vi "Image Marked Areas.vi"(7 "Calling VI Ref":refnum<vi>) -> ()   [LabVIEW 2016]
uses:
  <vilib>/Utility/miscctls.llb/LVPointTypeDef.ctl
  IMA Type Defs/IMA Actions.ctl
  Orca Flash Capture Manager/Orca Flash Capture Manager Controls/Orca Flash Capture Notifier Type.ctl
  Orca Flash Capture Manager/Orca Flash Capture Manager Controls/Orca Flash Capture Actions.ctl
  Orca Flash Capture Manager/Orca Flash Capture Manager Controls/Orca Flash Capture Switch Line Scan Modes.ctl
  Hardware Configuration/Hardware Configuration Controls/Device Function.ctl
  Hardware Configuration/Hardware Configuration Controls/Device Type.ctl
  IMA Type Defs/IMA Marked Positions.ctl
  Wide Field Drift Correction/WFDC Controls/WFDC Notifier Element.ctl
  Wide Field Drift Correction/WFDC Controls/WFDC Actions.ctl
  <vilib>/vision/Image Controls.llb/IMAQ Image.ctl
  Wide Field Drift Correction/WFDC Controls/WFDC External Sync.ctl
  Wide Field Drift Correction/WFDC Controls/WFDC Cycle Pause.ctl
  Wide Field Drift Correction/WFDC Controls/WFDC Status.ctl
  Device Library/Stages/Stages Controls/Stage Actions.ctl
  <vilib>/Utility/error.llb/whitespace.ctl
panel:
  in  "Capture":bool
  in  "Clear All":bool
  in  "Clear Selected":bool
  in  "Mark Point":bool
  in  "Marked Positions":i32(listbox)
  in  "Quit":bool
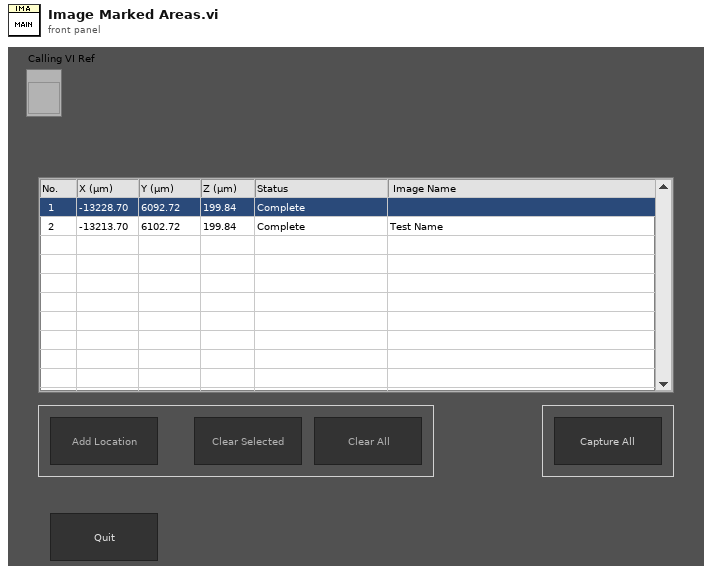
[diagram p1: front panel]
types:
  T1 = typedef "Orca Flash Capture Notifier Type.ctl" = cluster{"Actions":T2, "Running?":bool, "Preview Exposure (s)":dbl, "Capture Exposure (s)":dbl, "Cycles":u16, "Frames":u32, "No. of Z Steps":u16, "Z Step Size (µm)":dbl, "Base Path":path, "Init Z Position (µm)":dbl, "Lasers Lines":string[], "Save Path":path, "Line Scan?":bool, "Line Scan Mode":T3, "Collect Metadata?":bool, "channelCode":u8, "setupName":string}
  T2 = typedef "Orca Flash Capture Actions.ctl" = enum16{"Idle", "Live Preview", "Capture", "Check File Name", "Laser On", "Laser Off", "Open Shutters", "Close Shutters", "Set Exposure Time", "Start Acquisition", "Update SubFolder", "Write Metadata", "Setup", "Camera", "Switch", "Step", "Cycle", "External Cycle Sync", "Abort", "Quit"}
  T3 = typedef "Orca Flash Capture Switch Line Scan Modes.ctl" = enum32{"Automatic", "Use Presets", "Manual"}
  T4 = typedef "IMA Actions.ctl" = enum16{"Add Position", "Update Saved", "Remove Position", "Start Capture", "Move to Position", "Update Name", "Capture", "Switch", "Clear All", "Abort", "Exit Loop", "Quit"}
  T5 = enum16{"Always On", "Always Off", "Off While Running"}
  T6 = typedef "LVPointTypeDef.ctl" = cluster{"Horizontal":i16, "Vertical":i16}
  T7 = enum8{"Enabled", "Disabled", "Disabled and Grayed Out"}
  T8 = typedef "Device Function.ctl" = enum16{"Primary", "Secondary", "Overview", "Wide Field Drift Correction", "642 nm Excitation", "560 nm Excitation", "940 nm Excitation", "546 nm Excitation", "488 nm Excitation", "405 nm Excitation", "Objective Drift Correction", "4Pi Objective Lock", "Objective XY", "Objective Z", "Sample XY", "Sample Coarse Z", "Sample Z", "4Pi Lower", "4Pi Upper", "Mojo", "Adj Cavity", "Line Scanning", "Alert"}
  T9 = typedef "Device Type.ctl" = enum16{"AOTF", "Camera", "Deformable Mirror", "Laser", "Shutter", "Stage", "Waveform", "FPGA", "Email", "Filter Wheel"}
  T10 = typedef "WFDC External Sync.ctl" = cluster{"Cycle Sync":T11, "Z Offset":dbl, "WFDC Status":T12}
  T11 = typedef "WFDC Cycle Pause.ctl" = enum16{"Pause Requested", "Paused", "Resume Requested", "Resumed"}
  T12 = typedef "WFDC Status.ctl" = enum16{"Idle", "Busy", "DC Active", "Error", "Canceled"}
  T13 = typedef "WFDC Notifier Element.ctl" = cluster{"WFDC Actions":T14, "Initial XYZ Positions":dbl[], "Ref Images":T15[], "Calibration (slope, inter)":dbl[], "Log Drift?":bool, "Save WF Images?":bool, "Drift Image File Ref":refnum<file>, "Drift Positions File Ref":refnum<file>, "Base Path":path, "Latest Scan Path":path, "Error":errorcluster}
  T14 = typedef "WFDC Actions.ctl" = enum16{"Error Check", "Remote Start", "Find Focus", "Pre Correct Z", "Pre Correct XY", "Setup New DC", "Setup Camera", "Get Ref Images", "Calc Calibration", "Setup Data Log", "Switch Tabs", "Get Drift / Correct Z", "Correct XY Drift", "Start Cycle", "Stop DC", "Abort Remote", "Exit Loop", "Set Error", "Generate Calibration", "Quit"}
  T15 = typedef "IMAQ Image.ctl" = refnum<image>
  T16 = typedef "IMA Marked Positions.ctl" = cluster{"XYZ Positions":string[][], "File Paths":string[]}
  T17 = enum32{"Invalid", "Standard", "Closed", "Hidden", "Minimized", "Maximized"}
  T18 = typedef "Stage Actions.ctl" = enum16{"Get Position", "MVR", "MOVE", "HALT", "ONTARGET", "ERROR", "REFERENCE", "INIT", "VELOCITY", "STATUS", "EXIT", "HOME", "ZEROPOS", "NANOPOS", "ANALOG", "QUIT"}
  T19 = typedef "whitespace.ctl" = u16
  T20 = typedef "LVRectTypeDef.ctl" = cluster{"Left":i16, "Top":i16, "Right":i16, "Bottom":i16}
  T21 = typedef "LVBoundsTypeDef.ctl" = cluster{"Width":u32, "Height":u32}
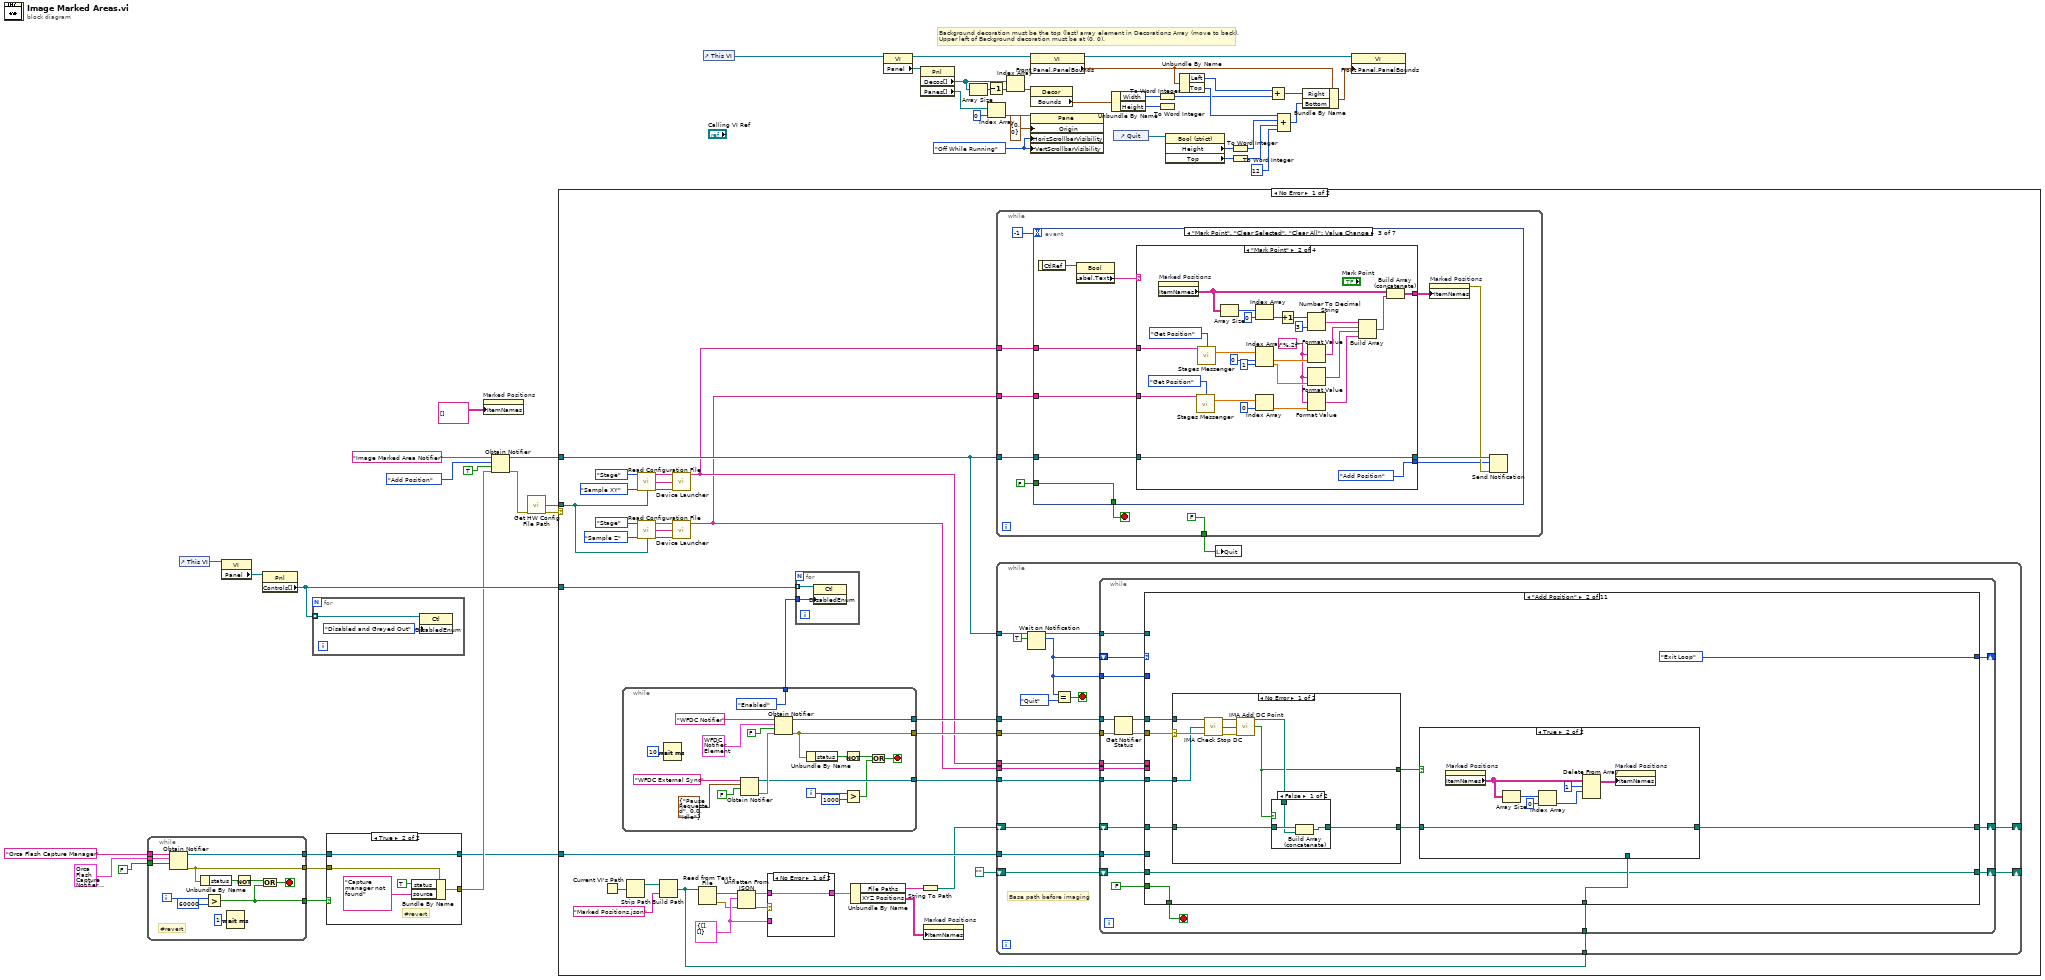
[diagram p0: block diagram]
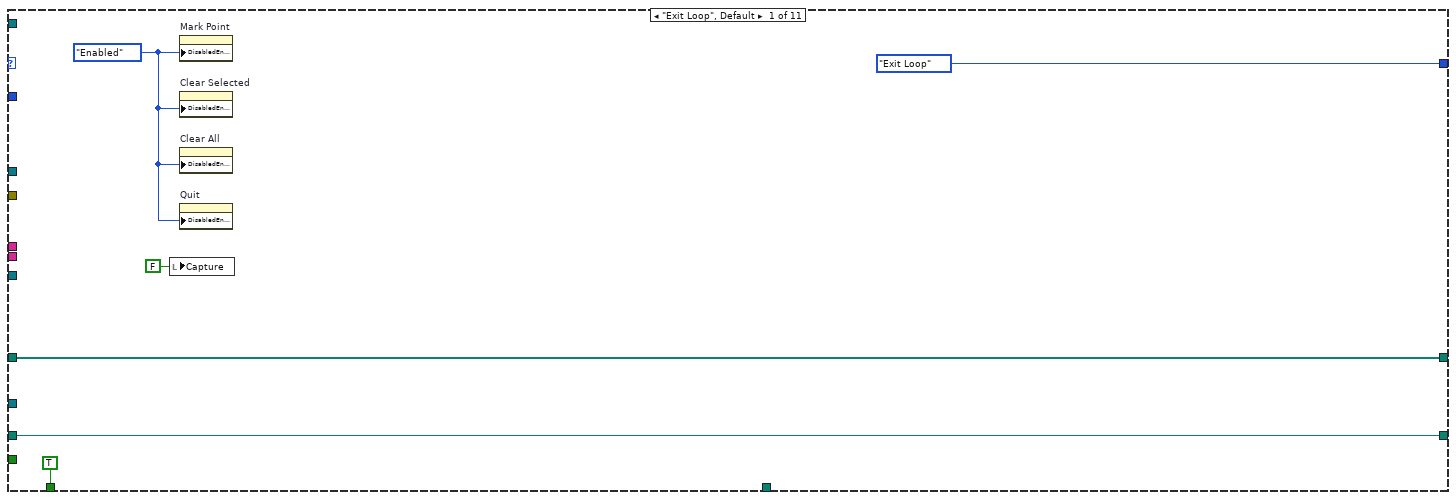
[diagram p4: hidden frame]
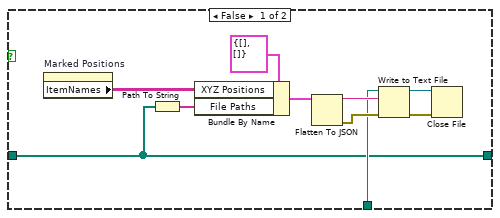
[diagram p5: hidden frame]
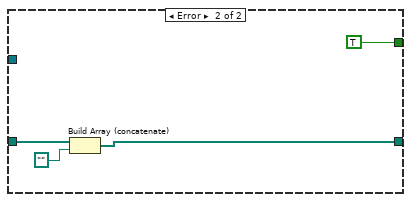
[diagram p7: hidden frame]
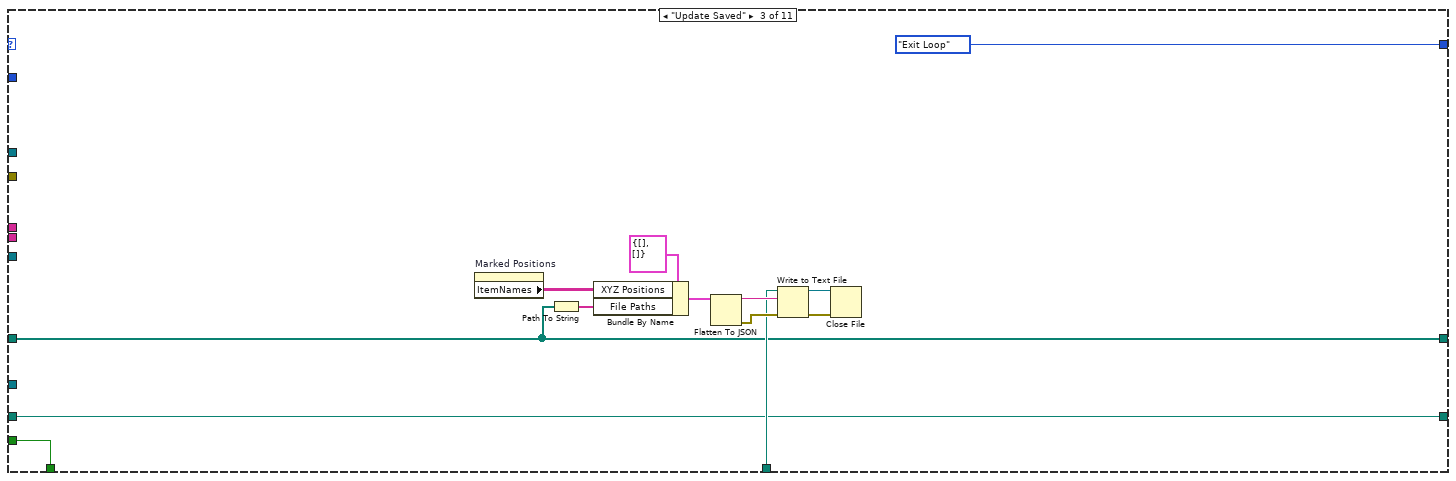
[diagram p8: hidden frame]
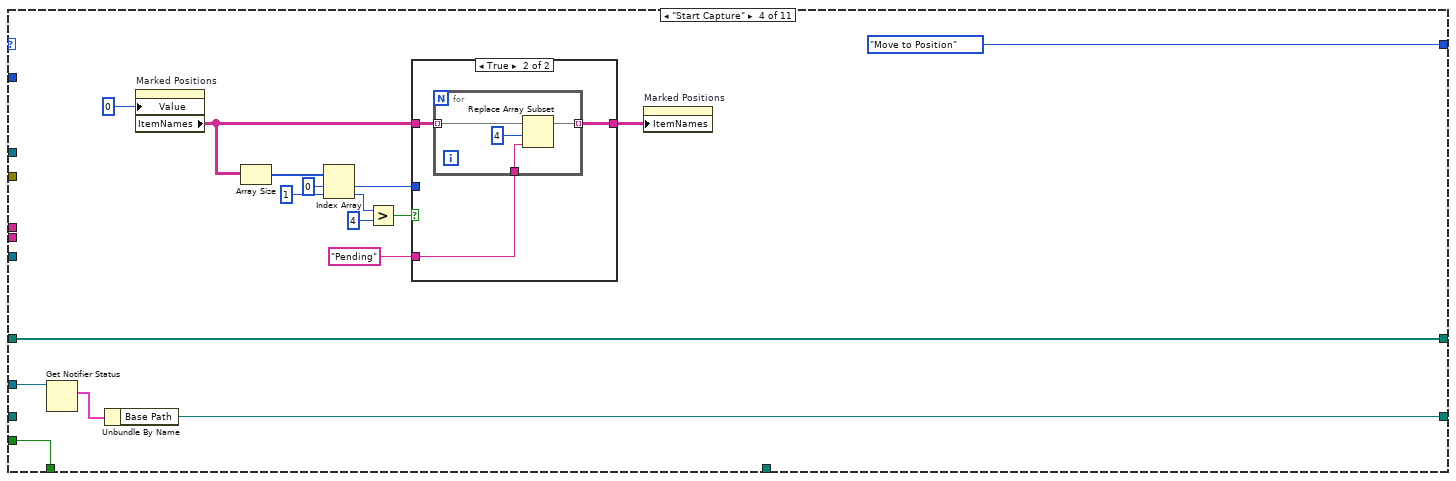
[diagram p9: hidden frame]
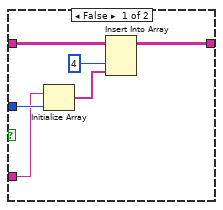
[diagram p10: hidden frame]
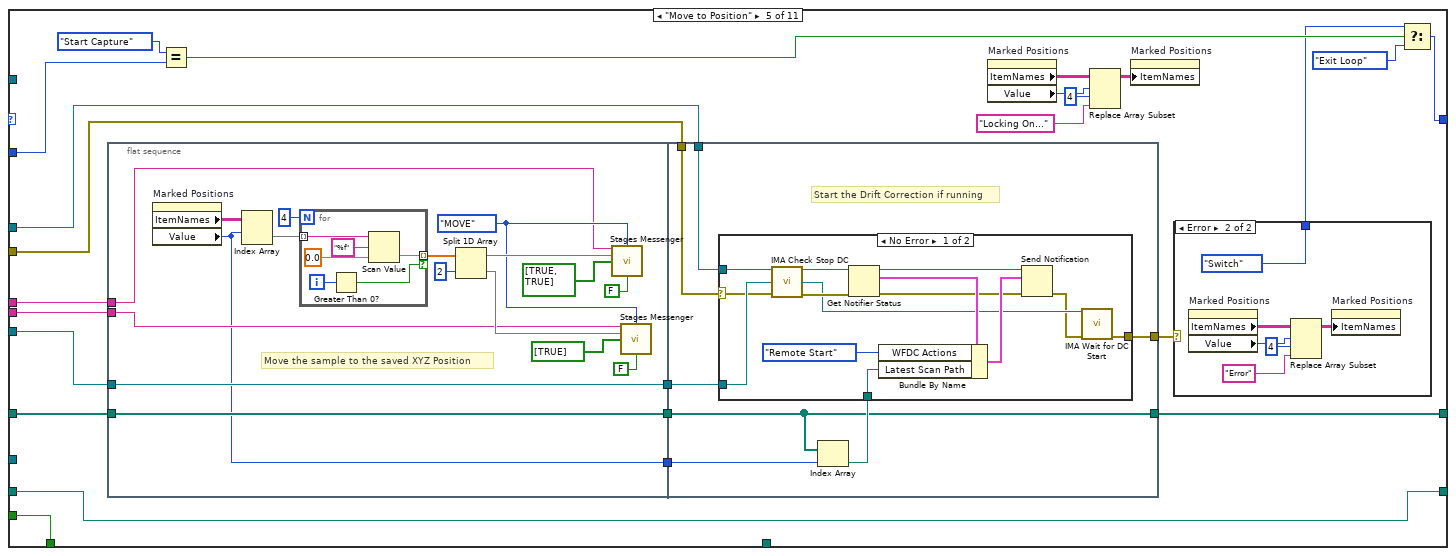
[diagram p11: hidden frame]
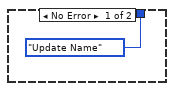
[diagram p12: hidden frame]
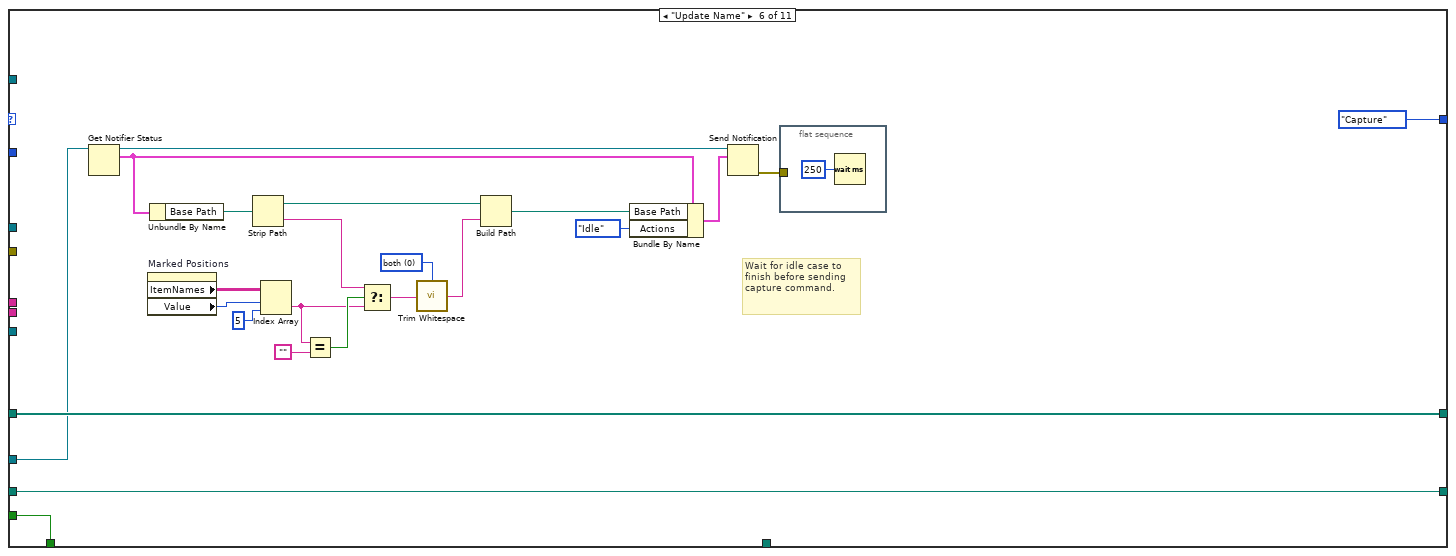
[diagram p14: hidden frame]
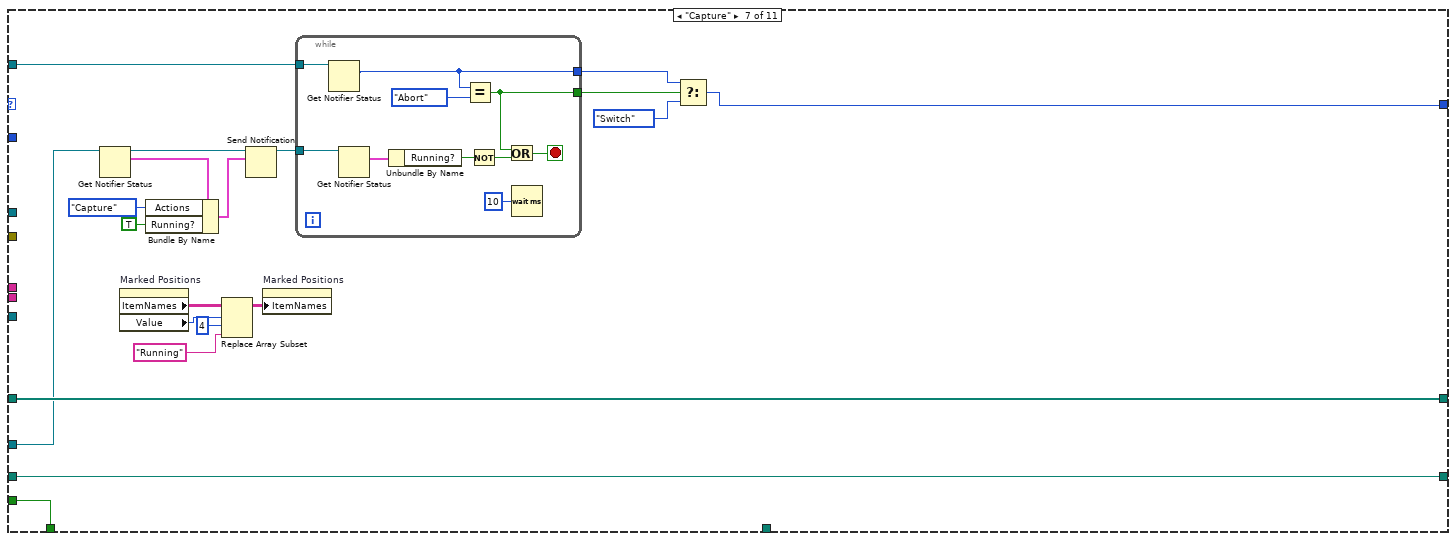
[diagram p15: hidden frame]
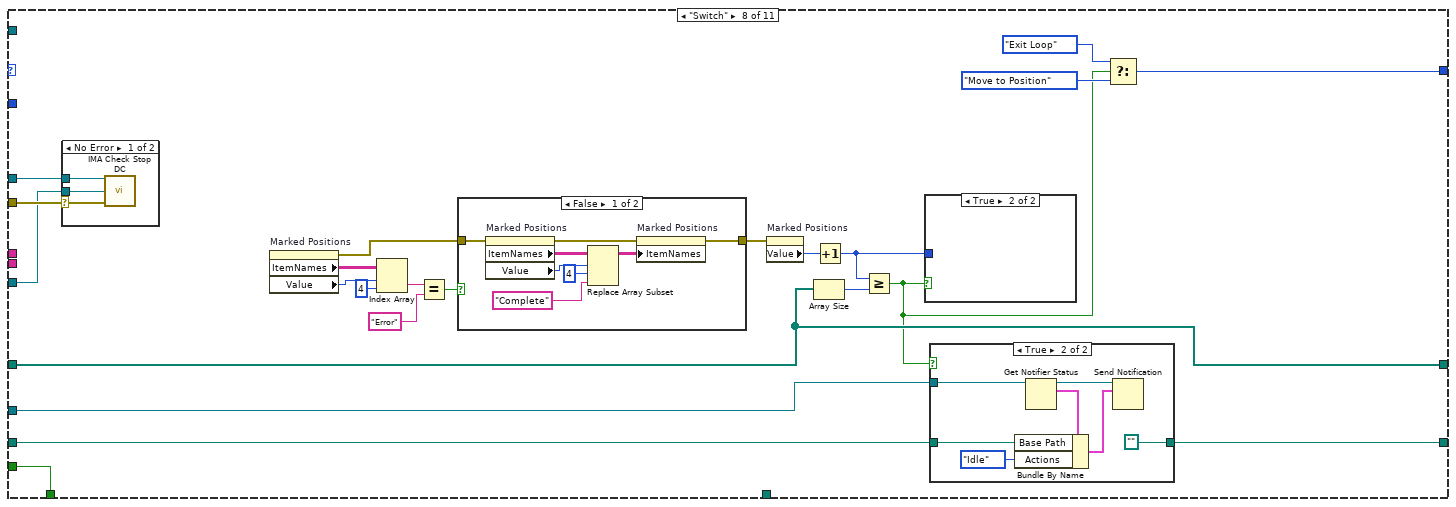
[diagram p16: hidden frame]
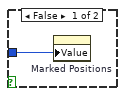
[diagram p20: hidden frame]
diagram:
  w29 = T5."Off While Running" ("Vertical Scrollbar Visibility")
  # "Background decoration must be the top (last) array element in Decorations Array (move to back).\nUpper left of Background decoration must be at (0, 0)."
  n1 = while {
    tunnel: FALSE ("create if not found? (T)") -> [w60]
    tunnel: "Orca Flash Capture Manager" ("name (unnamed)") -> [w59]
    tunnel: T1 {"Actions"=enum."Live Preview", "Running?"=FALSE, "Preview Exposure (s)"=0.1, "Capture Exposure (s)"=0.1, "Cycles"=1, "Frames"=0, "No. of Z Steps"=0, "Z Step Size (µm)"=0.0, "Base Path"=path "", "Init Z Position (µm)"=0.0, "Lasers Lines"=[], "Save Path"=path "", "Line Scan?"=FALSE, "Line Scan Mode"=enum."Automatic", "Collect Metadata?"=FALSE, "channelCode"=0, "setupName"=""} ("4Pi Capture Notifier Type") -> [w58]
    tunnel: [w54] -> w4
    tunnel: [w51] -> w5
    tunnel: [w49] -> w3
    i -> [w57]
    stop <- w50 stop-if-true
    # "#revert"
    n2 = Obtain Notifier(name (unnamed)=w59, notification data type=w58, create if not found? (T)=w60) -> (notifier out=w54:refnum<notifier>, error out=w49:errorcluster)  [unwired: 1 in, 1 out]
    n3 = Unbundle By Name(w49) -> ("status"=w53:bool)
    n4 = Greater?(x=w57, y=60000) -> (0:w51:bool)
    n5 = Wait (ms)(milliseconds to wait=u32 1) -> ()  [unwired: 1 out]
    n6 = Not(x=w53) -> (.not. x?=w52:bool)
    n7 = Or(x=w52, y=w51) -> (x .or. y?=w50:bool)
  }
  n8 = control-ref of="This VI"() -> (w11:refnum<vi>)
  n9 = property class="VI"(reference=w11) -> ("Panel"=w10:refnum<vi>)  [unwired: 1 in, 2 out]
  n10 = property class="Pnl"(reference=w10) -> ("Controls[]"=w9:refnum<vi>[])  [unwired: 1 in, 2 out]
  n11 = for {
    tunnel: w9 -> [w62] mode=indexing
    n12 = property class="Ctl"(reference=w62, "DisabledEnum"=T7."Disabled and Grayed Out" ("Disabled")) -> ()  [unwired: 1 in, 2 out]
  }
  n13 = case shown="True" w5 {
    tunnel: [w64 w67] -> w2
    tunnel: w4 -> [w63 w66]
    tunnel: [w63 w66] -> w1
    tunnel: w3 -> [w64 w65]
    frame False {
    }
    frame True {
      # "#revert"
      n14 = Bundle By Name(cluster=w65, "status"=TRUE, "source"="Capture manager not found") -> (w67:errorcluster)
    }
  }
  n15 = property on="Marked Positions" class="MCListbox (strict)"("ItemNames"=string[][] [] ("Item Names")) -> ()  [unwired: 2 in, 2 out]
  n16 = Obtain Notifier(name (unnamed)="Image Marked Area Notifier", notification data type=IMA_Actions."Add Position" ("Actions"), create if not found? (T)=TRUE, error in (no error)=w2) -> (notifier out=w13:refnum<notifier>, error out=w14:errorcluster)  [unwired: 1 out]
  n17 = call "Get HW Config File Path.vi"("Error"=w14) -> ("File Path"=w47:path, "Error"=w48:errorcluster)  [unwired: 13 in]
  n18 = case shown="No Error" w48 {
    selector: w48 -> [_ w585]
    tunnel: w47 -> [w93 _]
    tunnel: w13 -> [w92 w586]
    tunnel: w9 -> [w86 _]
    tunnel: w1 -> [w84 _]
    frame No Error {
      w80 = T16 {"XYZ Positions"=[], "File Paths"=[]} ("Marked Positions")
      n19 = Current VI's Path() -> (path=w79:path)
      n20 = while {
        tunnel: [w123] -> w91
        tunnel: [w111] -> w90
        tunnel: [w118] -> w89
        tunnel: [T7."Enabled" ("Disabled")] -> w85
        i -> [w116]
        stop <- w110 stop-if-true
        n21 = Wait (ms)(milliseconds to wait=u32 10) -> ()  [unwired: 1 out]
        n22 = Obtain Notifier(name (unnamed)="WFDC External Sync", notification data type=T10 {"Cycle Sync"=enum."Pause Requested", "Z Offset"=0.0, "WFDC Status"=enum."Idle"} ("WFDC External Sync"), create if not found? (T)=FALSE) -> (notifier out=w118:refnum<notifier>, error out=w119:errorcluster)  [unwired: 1 in, 1 out]
        n23 = Obtain Notifier(name (unnamed)="WFDC Notifier", notification data type=T13 {"WFDC Actions"=enum."Error Check", "Initial XYZ Positions"=[], "Ref Images"=[], "Calibration (slope, inter)"=[], "Log Drift?"=FALSE, "Save WF Images?"=FALSE, "Drift Image File Ref"=refnum, "Drift Positions File Ref"=refnum, "Base Path"=path "", "Latest Scan Path"=path "", "Error"={"status"=FALSE, "code"=0, "source"=""}} ("WFDC Notifier Element"), create if not found? (T)=FALSE, error in (no error)=w119) -> (notifier out=w123:refnum<notifier>, error out=w111:errorcluster)  [unwired: 1 out]
        n24 = Unbundle By Name(w111) -> ("status"=w114:bool)
        n25 = Not(x=w114) -> (.not. x?=w113:bool)
        n26 = Greater?(x=w116, y=1000) -> (0:w112:bool)
        n27 = Or(x=w113, y=w112) -> (x .or. y?=w110:bool)
      }
      n28 = Strip Path(path=w79) -> (stripped path=w73:path)  [unwired: 1 out]
      n29 = call "Read Configuration File.vi"("Device Type"=Device_Type."Stage", "Device Function"=Device_Function."Sample XY", "Config File Path"=w93) -> ("Unique Notifier Name"=w102:string, "Device Ports/IDs/Channels"=w104:string[], "Device Engine Path"=w103:path)  [unwired: 9 in, 1 out]
      n30 = call "Read Configuration File.vi"("Device Type"=Device_Type."Stage", "Device Function"=Device_Function."Sample Z", "Config File Path"=w93) -> ("Unique Notifier Name"=w96:string, "Device Ports/IDs/Channels"=w94:string[], "Device Engine Path"=w95:path)  [unwired: 9 in, 1 out]
      n31 = Build Path(base path=w73, name or relative path="Marked Positions.json") -> (appended path=w71:path)
      n32 = call "Device Launcher.vi"("Notifier Name"=w102, "Device Ports/IDs/Channels"=w104, "Device Engine Path"=w103) -> ("Notifier Name"=w88:string)  [unwired: 11 in, 1 out]
      n33 = call "Device Launcher.vi"("Notifier Name"=w96, "Device Ports/IDs/Channels"=w94, "Device Engine Path"=w95) -> ("Notifier Name"=w87:string)  [unwired: 11 in, 1 out]
      n34 = Read from Text File(file (use dialog)=w71) -> (text=w75:string, error out=w76:errorcluster)  [unwired: 3 in, 2 out]
      n35 = Unflatten From JSON(JSON string=w75, type and defaults=w80, error in (no error)=w76) -> (value=w78:T16, error out=w77:errorcluster)  [unwired: 4 in]
      n36 = case shown="No Error" w77 {
        tunnel: w78 -> [w105 _]
        tunnel: [w105 w106] -> w81
        tunnel: w80 -> [_ w106]
        frame No Error {
        }
        frame Error {
        }
      }
      n37 = for {
        tunnel: w86 -> [w108] mode=indexing
        tunnel: w85 -> [w107]
        n38 = property class="Ctl"(reference=w108, "DisabledEnum"=w107) -> ()  [unwired: 1 in, 2 out]
      }
      n39 = Unbundle By Name(w81) -> ("File Paths"=w83:string[], "XYZ Positions"=w82:string[][])
      n40 = String To Path(string=w83) -> (path=w72:path[])
      n41 = property on="Marked Positions" class="MCListbox (strict)"("ItemNames"=w82) -> ()  [unwired: 2 in, 2 out]
      n42 = while {
        tunnel: [FALSE] -> w99
        tunnel: w88 -> [w483]
        tunnel: w87 -> [w482]
        tunnel: w92 -> [w481]
        stop <- w485 stop-if-true
        n43 = event shown="[2] \"Mark Point\", \"Clear Selected\", \"Clear All\": Value Change" {
          selector: _ -> [_ _ _ _ _ _ _]
          dyn-events: _ -> [_ _ _ _ _ _ _]
          timeout: -1 -> [_ _ _ _ _ _ _]
          tunnel: FALSE -> [w488 w492 w503 w562 w567 w576 _]
          tunnel: [w488 w492 w503 w562 w567 w576 w579] -> w485
          tunnel: w483 -> [_ _ w500 _ _ _ _]
          tunnel: w482 -> [_ _ w499 _ _ _ _]
          tunnel: w481 -> [_ _ w497 w561 w565 w575 w578]
          event Timeout {
            n44 = event-data() -> ()  [unwired: 1 in, 1 out]
          }
          event Application Instance Close? {
            n45 = event-data() -> ()  [unwired: 1 in, 1 out]
            n46 = control-ref of="This VI"() -> (w489:refnum<vi>)
            n47 = invoke class="VI" method="FP.Open"(reference=w489, "Activate"=TRUE ("Activate?"), "State"=T17."Standard") -> ()  [unwired: 2 in, 5 out]
            n48 = event-data("Discard?"=TRUE) -> ()  [unwired: 1 in, 1 out]
          }
          event "Mark Point", "Clear Selected", "Clear All": Value Change {
            n49 = event-data() -> ("CtlRef"=w502:refnum<vi>)  [unwired: 1 in]
            n50 = property class="Bool"(reference=w502) -> ("Label.Text"=w498:string)  [unwired: 1 in, 2 out]
            n51 = case shown="\"Mark Point\"" w498 {
              tunnel: [w506 w518 w542 w552] -> w501
              tunnel: w500 -> [_ w516 _ _]
              tunnel: w499 -> [_ w513 _ _]
              tunnel: w497 -> [w505 w508 w539 w547]
              tunnel: [w505 w508 w535 w547] -> w496
              tunnel: [IMA_Actions."Exit Loop" ("notification") IMA_Actions."Add Position" ("notification") IMA_Actions."Exit Loop" ("notification") w546] -> w494
              frame Default {
                n52 = property on="Marked Positions" class="MCListbox (strict)"() -> ("ItemNames"=w506:string[][])  [unwired: 2 in, 2 out]
              }
              frame "Mark Point" {
                w515 = "%.2f" ("format string")
                n53 = property on="Marked Positions" class="MCListbox (strict)"() -> ("ItemNames"=w520:string[][])  [unwired: 2 in, 2 out]
                n54 = call "Stages Messenger.vi"("Stage Notifier Name"=w513, "Actions"=Stage_Actions."Get Position") -> ("Positions"=w512:dbl[])  [unwired: 10 in, 3 out]
                n55 = call "Stages Messenger.vi"("Stage Notifier Name"=w516, "Actions"=Stage_Actions."Get Position") -> ("Positions"=w517:dbl[])  [unwired: 10 in, 3 out]
                n56 = Array Size(array=w520) -> (size(s)=w526:i32[])
                n57 = Index Array(array=w526, index=0) -> (element=w524:i32)
                n58 = Index Array(array=w517, index #1=0 ("index"), index #2=1 ("index")) -> (element #1=w530:dbl, element #2=w529:dbl)
                n59 = Index Array(array=w512, index=0) -> (element=w510:dbl)
                n60 = Increment(x=w524) -> (x+1=w528:i32)
                n61 = Number To Decimal String(number=w528, width (-)=i16 3) -> (decimal integer string=w523:string)
                n62 = Format Value(format string=w515, value (0)=w530) -> (output string=w521:string)  [unwired: 1 in]
                n63 = Format Value(format string=w515, value (0)=w529) -> (output string=w522:string)  [unwired: 1 in]
                n64 = Format Value(format string=w515, value (0)=w510) -> (output string=w509:string)  [unwired: 1 in]
                n65 = Build Array(w523, w521, w522, w509) -> (w519:string[])
                n66 = Build Array (concatenate)(w520, w519) -> (w518:string[][])
              }
              frame "Clear Selected" {
                n67 = Send Notification(notification=IMA_Actions."Remove Position", notifier=w539) -> (notifier out=w535:refnum<notifier>, error out=w537:errorcluster)  [unwired: 1 in]
                n68 = flat-sequence {
                  tunnel: w537 -> [w544]
                  tunnel: [w544] -> w536
                  frame #0 {
                    n69 = Wait (ms)(milliseconds to wait=u32 20) -> ()  [unwired: 1 out]
                  }
                }
                n70 = property on="Marked Positions" class="MCListbox (strict)"() -> ("ItemNames"=w543:string[][])  [unwired: 2 in, 2 out]
                n71 = property on="Marked Positions" class="MCListbox (strict)"(error in=w536) -> ("Value"=w540:i32)  [unwired: 1 in, 2 out]
                n72 = Delete From Array(array=w543, length=1, index (row)=w540) -> (array with subset deleted=w542:string[][])  [unwired: 1 in, 1 out]
              }
              frame "Clear All" {
                n73 = Two Button Dialog(message="Clear all marked positions?", 1:"Cancel" ("F button name (\"Cancel\")"), 2:"Okay" ("T button name (\"OK\")")) -> (T button?=w548:bool)
                n74 = case shown="False" w548 {
                  tunnel: [w554 string[][] []] -> w552
                  tunnel: [IMA_Actions."Exit Loop" ("notification") IMA_Actions."Clear All" ("notification")] -> w546
                  frame False {
                    n75 = property on="Marked Positions" class="MCListbox (strict)"() -> ("ItemNames"=w554:string[][])  [unwired: 2 in, 2 out]
                  }
                  frame True {
                  }
                }
              }
            }
            n76 = property on="Marked Positions" class="MCListbox (strict)"("ItemNames"=w501) -> (error out=w495:errorcluster)  [unwired: 2 in, 1 out]
            n77 = Send Notification(notification=w494, notifier=w496, error in (no error)=w495) -> ()  [unwired: 2 out]
          }
          event "Marked Positions": Double Click {
            n78 = event-data() -> ()  [unwired: 1 in, 1 out]
            n79 = Two Button Dialog(message="Move to marked position?", 1:"Cancel" ("F button name (\"Cancel\")"), 2:"Yes" ("T button name (\"OK\")")) -> (T button?=w557:bool)
            n80 = case shown="True" w557 {
              tunnel: w561 -> [_ w564]
              frame False {
              }
              frame True {
                n81 = Send Notification(notification=IMA_Actions."Move to Position", notifier=w564) -> ()  [unwired: 1 in, 2 out]
              }
            }
          }
          event "Marked Positions": Edit Cell {
            n82 = event-data() -> ()  [unwired: 1 in, 6 out]
            n83 = Send Notification(notification=IMA_Actions."Update Saved", notifier=w565) -> ()  [unwired: 1 in, 2 out]
          }
          event "Capture": Value Change {
            n84 = event-data() -> ("NewVal"=w572:bool)  [unwired: 1 in]
            n85 = Select(t=IMA_Actions."Start Capture", s=w572, f=IMA_Actions."Abort" ("y")) -> (s? t:f=w573:T4)
            n86 = Select(t=T7."Disabled and Grayed Out" ("Disabled"), s=w572, f=T7."Enabled" ("Disabled")) -> (s? t:f=w569:T7)
            n87 = Send Notification(notification=w573, notifier=w575) -> ()  [unwired: 1 in, 2 out]
            n88 = property on="Mark Point" class="Bool"("DisabledEnum"=w569) -> ()  [unwired: 2 in, 2 out]
            n89 = property on="Clear Selected" class="Bool"("DisabledEnum"=w569) -> ()  [unwired: 2 in, 2 out]
            n90 = property on="Clear All" class="Bool"("DisabledEnum"=w569) -> ()  [unwired: 2 in, 2 out]
            n91 = property on="Quit" class="Bool (strict)"("DisabledEnum"=w569) -> ()  [unwired: 2 in, 2 out]
          }
          event "Quit": Value Change {
            n92 = event-data() -> ("NewVal"=w579:bool)  [unwired: 1 in]
            n93 = Send Notification(notification=IMA_Actions."Quit", notifier=w578) -> ()  [unwired: 1 in, 2 out]
          }
        }
      }
      n94 = while {
        tunnel: w92 -> [w143]
        tunnel: w91 -> [w137]
        tunnel: w90 -> [w136]
        tunnel: w89 -> [w138]
        shift-right: [w134] -> _
        shift-left: w72 -> [w135]
        tunnel: w88 -> [w132]
        tunnel: w87 -> [w131]
        tunnel: w84 -> [w130]
        tunnel: w71 -> [w129]
        shift-right: [w128] -> _
        shift-left: path "" -> [w127]
        stop <- w140 stop-if-true
        # "Base path before imaging"
        n95 = Wait on Notification(notifier=w143, ignore previous (F)=TRUE) -> (notifier out=w139:refnum<notifier>, notification=w133:T4)  [unwired: 2 in, 2 out]
        n96 = Equal?(x=w133, y=IMA_Actions."Quit") -> (x = y?=w140:bool)
        n97 = while {
          shift-right: [w158] -> _
          shift-left: w133 -> [w161]
          tunnel: w139 -> [w162]
          tunnel: w138 -> [w157]
          tunnel: w137 -> [w156]
          tunnel: w136 -> [w155]
          shift-right: [w151] -> w134
          shift-left: w135 -> [w152]
          tunnel: w133 -> [w150]
          tunnel: w132 -> [w149]
          tunnel: w131 -> [w148]
          tunnel: w130 -> [w147]
          tunnel: w129 -> [w146]
          shift-right: [w145] -> w128
          shift-left: w127 -> [w144]
          stop <- w159 stop-if-true
          n98 = Get Notifier Status(notifier=w156, error in (no error)=w155) -> (notifier out=w154:refnum<notifier>, error out=w153:errorcluster)  [unwired: 3 out]
          n99 = case shown="\"Add Position\"" w161 {
            tunnel: w162 -> [_ _ _ _ _ _ w359 _ _ _ w473]
            tunnel: w154 -> [_ w176 _ _ w274 _ _ w403 _ _ w476]
            tunnel: w153 -> [_ w177 _ _ w275 _ _ w402 _ _ w474]
            tunnel: [TRUE w179 w227 w244 w281 w356 w377 w410 w448 w466 TRUE] -> w159
            tunnel: FALSE -> [_ w179 w227 w244 w281 w356 w377 w410 w448 w466 _]
            tunnel: [IMA_Actions."Exit Loop" ("y") IMA_Actions."Exit Loop" ("y") IMA_Actions."Exit Loop" ("y") IMA_Actions."Move to Position" ("y") w265 IMA_Actions."Capture" ("y") w371 w404 IMA_Actions."Exit Loop" ("y") IMA_Actions."Exit Loop" ("y") IMA_Actions."Quit" ("y")] -> w158
            tunnel: w157 -> [_ w175 _ _ w276 _ _ w401 _ _ w475]
            tunnel: w152 -> [w167 w174 w216 w243 w279 w355 w376 w392 w445 _ w472]
            tunnel: [w167 w170 w216 w243 w278 w355 w376 w392 w437 w468 w472] -> w151
            tunnel: w150 -> [_ _ _ _ w269 _ _ _ _ _ _]
            tunnel: w149 -> [_ _ _ _ w272 _ _ _ _ _ _]
            tunnel: w148 -> [_ _ _ _ w273 _ _ _ _ _ _]
            tunnel: w147 -> [_ _ _ w229 _ w353 w370 w391 _ _ _]
            tunnel: w146 -> [_ w172 w217 _ _ _ _ _ w433 w460 _]
            tunnel: [w163 w171 w215 w228 w263 w336 w364 w388 w432 w459 w471] -> w145
            tunnel: w144 -> [w163 w171 w215 _ w263 w336 w364 w389 w432 w459 w471]
            frame "Exit Loop", Default {
              w165 = T7."Enabled" ("Disabled")
              n100 = local write "Capture"(FALSE ("Capture")) -> ()
              n101 = property on="Mark Point" class="Bool"("DisabledEnum"=w165) -> ()  [unwired: 2 in, 2 out]
              n102 = property on="Clear Selected" class="Bool"("DisabledEnum"=w165) -> ()  [unwired: 2 in, 2 out]
              n103 = property on="Clear All" class="Bool"("DisabledEnum"=w165) -> ()  [unwired: 2 in, 2 out]
              n104 = property on="Quit" class="Bool (strict)"("DisabledEnum"=w165) -> ()  [unwired: 2 in, 2 out]
            }
            frame "Add Position" {
              n105 = case shown="No Error" w177 {
                selector: w177 -> [w202 _]
                tunnel: w176 -> [w204 _]
                tunnel: w175 -> [w201 _]
                tunnel: w174 -> [w206 w214]
                tunnel: [w205 w213] -> w173
                tunnel: [w197 TRUE ("Canceled")] -> w169
                frame No Error {
                  n106 = call "IMA Check Stop DC.vi"("WFDC Notifier"=w204, "WFDC External Sync"=w201, "Error"=w202) -> ("WFDC Notifier (Dup)"=w203:refnum<notifier>, "WFDC External Sync (Dup)"=w199:refnum<notifier>, "Error Out"=w200:errorcluster)  [unwired: 10 in]
                  n107 = call "IMA Add DC Point.vi"("WFDC Notifier"=w203, "WFDC External Sync"=w199, "Error"=w200) -> ("Scan Path"=w198:path, "Canceled"=w197:bool)  [unwired: 10 in, 1 out]
                  n108 = case shown="False" w197 {
                    tunnel: w206 -> [w209 w210]
                    tunnel: [w208 w210] -> w205
                    tunnel: w198 -> [w207 _]
                    frame False {
                      n109 = Build Array (concatenate)(w209, w207) -> (w208:path[])
                    }
                    frame True {
                    }
                  }
                }
                frame Error {
                  n110 = Build Array (concatenate)(w214, path "") -> (w213:path[])
                }
              }
              n111 = case shown="True" w169 {
                tunnel: w173 -> [w180 w196]
                tunnel: w172 -> [w181 _]
                tunnel: [w180 w196] -> w170
                frame False {
                  n112 = property on="Marked Positions" class="MCListbox (strict)"() -> ("ItemNames"=w188:string[][])  [unwired: 2 in, 2 out]
                  n113 = Path To String(path=w180) -> (string=w187:string[])
                  n114 = Bundle By Name(cluster=T16 {"XYZ Positions"=[], "File Paths"=[]} ("Marked Positions"), "XYZ Positions"=w188, "File Paths"=w187) -> (w186:T16)
                  n115 = Flatten To JSON(anything=w186) -> (JSON string=w185:string, 11:w183:errorcluster)  [unwired: 2 in]
                  n116 = Write to Text File(file (use dialog)=w181, text=w185, error in=w183) -> (refnum out=w184:refnum<file>, error out=w182:errorcluster)  [unwired: 1 in, 1 out]
                  n117 = Close File(refnum=w184, error in=w182) -> ()  [unwired: 2 out]
                }
                frame True {
                  n118 = property on="Marked Positions" class="MCListbox (strict)"() -> ("ItemNames"=w194:string[][])  [unwired: 2 in, 2 out]
                  n119 = Array Size(array=w194) -> (size(s)=w193:i32[])
                  n120 = Index Array(array=w193, index=0) -> (element=w191:i32)
                  n121 = Delete From Array(array=w194, length=1, index (row)=w191) -> (array with subset deleted=w190:string[][])  [unwired: 1 in, 1 out]
                  n122 = property on="Marked Positions" class="MCListbox (strict)"("ItemNames"=w190) -> ()  [unwired: 2 in, 2 out]
                }
              }
            }
            frame "Update Saved" {
              n123 = property on="Marked Positions" class="MCListbox (strict)"() -> ("ItemNames"=w224:string[][])  [unwired: 2 in, 2 out]
              n124 = Path To String(path=w216) -> (string=w223:string[])
              n125 = Bundle By Name(cluster=T16 {"XYZ Positions"=[], "File Paths"=[]} ("Marked Positions"), "XYZ Positions"=w224, "File Paths"=w223) -> (w222:T16)
              n126 = Flatten To JSON(anything=w222) -> (JSON string=w221:string, 11:w219:errorcluster)  [unwired: 2 in]
              n127 = Write to Text File(file (use dialog)=w217, text=w221, error in=w219) -> (refnum out=w220:refnum<file>, error out=w218:errorcluster)  [unwired: 1 in, 1 out]
              n128 = Close File(refnum=w220, error in=w218) -> ()  [unwired: 2 out]
            }
            frame "Start Capture" {
              n129 = Get Notifier Status(notifier=w229) -> (current notification=w230:T1)  [unwired: 1 in, 4 out]
              n130 = Unbundle By Name(w230) -> ("Base Path"=w228:path)
              n131 = property on="Marked Positions" class="MCListbox (strict)"("Value"=0 ("Focus Row")) -> ("ItemNames"=w233:string[][])  [unwired: 2 in, 2 out]
              n132 = Array Size(array=w233) -> (size(s)=w240:i32[])
              n133 = Index Array(array=w240, index #1=0 ("index"), index #2=1 ("index")) -> (element #1=w238:i32, element #2=w236:i32)
              n134 = Greater?(x=w236, y=4) -> (0:w234:bool)
              n135 = case shown="True" w234 {
                tunnel: w238 -> [w250 _]
                tunnel: w233 -> [w248 w253]
                tunnel: [w245 w252] -> w232
                tunnel: "Pending" -> [w249 w251]
                frame False {
                  n136 = Initialize Array(w249, w250) -> (w247:string[])
                  n137 = Insert Into Array(array=w248, index (col)=4 ("disabled index (col)"), new element=w247) -> (w245:string[][])  [unwired: 1 in]
                }
                frame True {
                  n138 = for {
                    tunnel: w253 -> [w257] mode=indexing
                    tunnel: [w255] -> w252 mode=indexing
                    tunnel: w251 -> [w254]
                    n139 = Replace Array Subset(array=w257, new element=w254, index=4) -> (w255:string[])
                  }
                }
              }
              n140 = property on="Marked Positions" class="MCListbox (strict)"("ItemNames"=w232) -> ()  [unwired: 2 in, 2 out]
            }
            frame "Move to Position" {
              n141 = flat-sequence {
                tunnel: [w294] -> w280
                tunnel: w279 -> [w294]
                tunnel: [w293] -> w277
                tunnel: w276 -> [w293]
                tunnel: w273 -> [w291]
                tunnel: w272 -> [w292]
                tunnel: [w290] -> w267
                tunnel: w280 -> [w317]
                tunnel: [w317] -> w278
                tunnel: w277 -> [w316]
                tunnel: w275 -> [w315]
                tunnel: w274 -> [w314]
                tunnel: w267 -> [w313]
                tunnel: [w312] -> w266
                frame #0 {
                  w295 = Stage_Actions."MOVE" ("Actions")
                  # "Move the sample to the saved XYZ Position"
                  n142 = property on="Marked Positions" class="MCListbox (strict)"() -> ("ItemNames"=w303:string[][], "Value"=w290:i32)  [unwired: 2 in, 2 out]
                  n143 = Index Array(array=w303, index (row)=w290) -> (element=w300:string[])  [unwired: 1 in]
                  n144 = for {
                    N: 4 -> [_]
                    tunnel: w300 -> [w309] mode=indexing
                    tunnel: [w308] -> w299 mode=indexing if=w306
                    i -> [w307]
                    n145 = Greater Than 0?(x=w307) -> (x > 0?=w306:bool)
                    n146 = Scan Value(string=w309, format string="%f", default (0 dbl)=0.0) -> (value=w308:dbl)  [unwired: 1 out]
                  }
                  n147 = Split 1D Array(array=w299, index=2) -> (first subarray=w297:dbl[], second subarray=w296:dbl[])
                  n148 = call "Stages Messenger.vi"("Stage Notifier Name"=w292, "Actions"=w295, "Setpoint"=w297, "Axis"=bool[] [TRUE, TRUE], "Exit While Busy?"=FALSE ("Wait for On Target? (F)")) -> ()  [unwired: 7 in, 4 out]
                  n149 = call "Stages Messenger.vi"("Stage Notifier Name"=w291, "Actions"=w295, "Setpoint"=w296, "Axis"=bool[] [TRUE], "Exit While Busy?"=FALSE ("Wait for On Target? (F)")) -> ()  [unwired: 7 in, 4 out]
                }
                frame #1 {
                  # "Start the Drift Correction if running"
                  n150 = Index Array(array=w317, index=w313) -> (element=w318:path)
                  n151 = case shown="No Error" w315 {
                    selector: w315 -> [w328 w333]
                    tunnel: w314 -> [w332 _]
                    tunnel: w316 -> [w331 _]
                    tunnel: w318 -> [w323 _]
                    tunnel: [w319 w333] -> w312
                    frame No Error {
                      n152 = call "IMA Check Stop DC.vi"("WFDC Notifier"=w332, "WFDC External Sync"=w331, "Error"=w328) -> ("WFDC Notifier (Dup)"=w330:refnum<notifier>, "WFDC External Sync (Dup)"=w321:refnum<notifier>, "Error Out"=w329:errorcluster)  [unwired: 10 in]
                      n153 = Get Notifier Status(notifier=w330, error in (no error)=w329) -> (notifier out=w327:refnum<notifier>, current notification=w326:T13, error out=w324:errorcluster)  [unwired: 2 out]
                      n154 = Bundle By Name(cluster=w326, "WFDC Actions"=WFDC_Actions."Remote Start", "Latest Scan Path"=w323) -> (w325:T13)
                      n155 = Send Notification(notification=w325, notifier=w327, error in (no error)=w324) -> (error out=w320:errorcluster)  [unwired: 1 out]
                      n156 = call "IMA Wait for DC Start.vi"("WFDC External Sync"=w321, "Error"=w320) -> ("Error Out"=w319:errorcluster)  [unwired: 12 in, 1 out]
                    }
                    frame Error {
                    }
                  }
                }
              }
              n157 = Equal?(x=IMA_Actions."Start Capture" ("y"), y=w269) -> (x = y?=w271:bool)
              n158 = property on="Marked Positions" class="MCListbox (strict)"() -> ("ItemNames"=w262:string[][], "Value"=w261:i32)  [unwired: 2 in, 2 out]
              n159 = Replace Array Subset(array=w262, new element="Locking On..." ("new element/subarray"), index (row)=w261, index (col)=4 ("disabled index (col)")) -> (w258:string[][])
              n160 = property on="Marked Positions" class="MCListbox (strict)"("ItemNames"=w258) -> ()  [unwired: 2 in, 2 out]
              n161 = case shown="Error" w266 {
                tunnel: [IMA_Actions."Update Name" ("t") IMA_Actions."Switch" ("y")] -> w264
                frame No Error {
                }
                frame Error {
                  n162 = property on="Marked Positions" class="MCListbox (strict)"() -> ("ItemNames"=w284:string[][], "Value"=w285:i32)  [unwired: 2 in, 2 out]
                  n163 = Replace Array Subset(array=w284, new element="Error" ("new element/subarray"), index (row)=w285, index (col)=4 ("disabled index (col)")) -> (w288:string[][])
                  n164 = property on="Marked Positions" class="MCListbox (strict)"("ItemNames"=w288) -> ()  [unwired: 2 in, 2 out]
                }
              }
              n165 = Select(t=w264, s=w271, f=IMA_Actions."Exit Loop" ("y")) -> (s? t:f=w265:T4)
            }
            frame "Update Name" {
              w350 = T19 0 items=["both", "start of string", "end of string"] ("location (both)")
              # "Wait for idle case to finish before sending capture command."
              n166 = Get Notifier Status(notifier=w353) -> (notifier out=w352:refnum<notifier>, current notification=w346:T1)  [unwired: 1 in, 3 out]
              n167 = property on="Marked Positions" class="MCListbox (strict)"() -> ("ItemNames"=w348:string[][], "Value"=w347:i32)  [unwired: 2 in, 2 out]
              n168 = Unbundle By Name(w346) -> ("Base Path"=w351:path)
              n169 = Strip Path(path=w351) -> (stripped path=w345:path, name=w339:string)
              n170 = Index Array(array=w348, index (row)=w347, index (col)=5 ("disabled index (col)")) -> (element=w338:string)
              n171 = Equal?(x=w338, y="") -> (x = y?=w340:bool)
              n172 = Select(t=w339, s=w340, f=w338) -> (s? t:f=w337:string)
              n173 = call <vilib>:"Trim Whitespace.vi"("string"=w337, "location (both)"=w350) -> ("trimmed string"=w344:string)
              n174 = Build Path(base path=w345, name or relative path=w344) -> (appended path=w343:path)
              n175 = Bundle By Name(cluster=w346, "Base Path"=w343, "Actions"=Orca_Flash_Capture_Actions."Idle") -> (w342:T1)
              n176 = Send Notification(notification=w342, notifier=w352) -> (error out=w334:errorcluster)  [unwired: 1 in, 1 out]
              n177 = flat-sequence {
                tunnel: w334 -> [_]
                frame #0 {
                  n178 = Wait (ms)(milliseconds to wait=u32 250) -> ()  [unwired: 1 out]
                }
              }
            }
            frame "Capture" {
              n179 = Get Notifier Status(notifier=w370) -> (notifier out=w373:refnum<notifier>, current notification=w375:T1)  [unwired: 1 in, 3 out]
              n180 = property on="Marked Positions" class="MCListbox (strict)"() -> ("ItemNames"=w365:string[][], "Value"=w366:i32)  [unwired: 2 in, 2 out]
              n181 = Bundle By Name(cluster=w375, "Actions"=Orca_Flash_Capture_Actions."Capture", "Running?"=TRUE) -> (w372:T1)
              n182 = Replace Array Subset(array=w365, new element="Running" ("new element/subarray"), index (row)=w366, index (col)=4 ("disabled index (col)")) -> (w369:string[][])
              n183 = Send Notification(notification=w372, notifier=w373) -> (notifier out=w358:refnum<notifier>)  [unwired: 1 in, 1 out]
              n184 = property on="Marked Positions" class="MCListbox (strict)"("ItemNames"=w369) -> ()  [unwired: 2 in, 2 out]
              n185 = while {
                tunnel: w358 -> [w387]
                tunnel: w359 -> [w385]
                tunnel: [w382] -> w362
                tunnel: [w380] -> w361
                stop <- w383 stop-if-true
                n186 = Get Notifier Status(notifier=w385) -> (current notification=w380:T4)  [unwired: 1 in, 4 out]
                n187 = Get Notifier Status(notifier=w387) -> (current notification=w386:T1)  [unwired: 1 in, 4 out]
                n188 = Unbundle By Name(w386) -> ("Running?"=w384:bool)
                n189 = Equal?(x=w380, y=IMA_Actions."Abort") -> (x = y?=w382:bool)
                n190 = Not(x=w384) -> (.not. x?=w381:bool)
                n191 = Or(x=w382, y=w381) -> (x .or. y?=w383:bool)
                n192 = Wait (ms)(milliseconds to wait=u32 10) -> ()  [unwired: 1 out]
              }
              n193 = Select(t=w361, s=w362, f=IMA_Actions."Switch") -> (s? t:f=w371:T4)
            }
            frame "Switch" {
              n194 = case shown="No Error" w402 {
                selector: w402 -> [w429 _]
                tunnel: w403 -> [w430 _]
                tunnel: w401 -> [w428 _]
                frame No Error {
                  n195 = call "IMA Check Stop DC.vi"("WFDC Notifier"=w430, "WFDC External Sync"=w428, "Error"=w429) -> ()  [unwired: 10 in, 3 out]
                }
                frame Error {
                }
              }
              n196 = property on="Marked Positions" class="MCListbox (strict)"() -> (error out=w400:errorcluster, "ItemNames"=w394:string[][], "Value"=w395:i32)  [unwired: 2 in, 1 out]
              n197 = Index Array(array=w394, index (row)=w395, index (col)=4 ("disabled index (col)")) -> (element=w397:string)
              n198 = Equal?(x=w397, y="Error") -> (x = y?=w399:bool)
              n199 = case shown="False" w399 {
                tunnel: w400 -> [w421 w427]
                tunnel: [w419 w427] -> w393
                frame False {
                  n200 = property on="Marked Positions" class="MCListbox (strict)"(error in=w421) -> (error out=w420:errorcluster, "ItemNames"=w422:string[][], "Value"=w423:i32)  [unwired: 1 in, 1 out]
                  n201 = Replace Array Subset(array=w422, new element="Complete" ("new element/subarray"), index (row)=w423, index (col)=4 ("disabled index (col)")) -> (w426:string[][])
                  n202 = property on="Marked Positions" class="MCListbox (strict)"(error in=w420, "ItemNames"=w426) -> (error out=w419:errorcluster)  [unwired: 1 in, 1 out]
                }
                frame True {
                }
              }
              n203 = property on="Marked Positions" class="MCListbox (strict)"(error in=w393) -> ("Value"=w409:i32)  [unwired: 1 in, 2 out]
              n204 = Array Size(array=w392) -> (size(s)=w408:i32)
              n205 = Increment(x=w409) -> (x+1=w407:i32)
              n206 = Greater Or Equal?(x=w407, y=w408) -> (x >= y?=w390:bool)
              n207 = case shown="True" w390 {
                tunnel: w407 -> [w431 _]
                frame False {
                  n208 = property on="Marked Positions" class="MCListbox (strict)"("Value"=w431) -> ()  [unwired: 2 in, 2 out]
                }
                frame True {
                }
              }
              n209 = case shown="True" w390 {
                tunnel: w391 -> [_ w418]
                tunnel: w389 -> [w411 w415]
                tunnel: [w411 path ""] -> w388
                frame False {
                }
                frame True {
                  n210 = Get Notifier Status(notifier=w418) -> (notifier out=w417:refnum<notifier>, current notification=w416:T1)  [unwired: 1 in, 3 out]
                  n211 = Bundle By Name(cluster=w416, "Base Path"=w415, "Actions"=Orca_Flash_Capture_Actions."Idle") -> (w414:T1)
                  n212 = Send Notification(notification=w414, notifier=w417) -> ()  [unwired: 1 in, 2 out]
                }
              }
              n213 = Select(t=IMA_Actions."Exit Loop" ("y"), s=w390, f=IMA_Actions."Move to Position" ("y")) -> (s? t:f=w404:T4)
            }
            frame "Remove Position" {
              n214 = property on="Marked Positions" class="MCListbox (strict)"() -> ("Value"=w447:i32)  [unwired: 2 in, 2 out]
              n215 = property on="Marked Positions" class="MCListbox (strict)"() -> ("ItemNames"=w436:string[][])  [unwired: 2 in, 2 out]
              n216 = Delete From Array(array=w445, length=1, index=w447) -> (array with subset deleted=w437:path[])  [unwired: 1 out]
              n217 = Array Size(array=w436) -> (size(s)=w435:i32[])
              n218 = while {
                tunnel: w435 -> [w458]
                tunnel: [w450] -> w434
                i -> [w456]
                stop <- w452 stop-if-true
                n219 = property on="Marked Positions" class="MCListbox (strict)"() -> ("ItemNames"=w450:string[][])  [unwired: 2 in, 2 out]
                n220 = Wait (ms)(milliseconds to wait=u32 2) -> ()  [unwired: 1 out]
                n221 = Array Size(array=w450) -> (size(s)=w457:i32[])
                n222 = Greater?(x=w456, y=500) -> (0:w454:bool)
                n223 = Not Equal?(x=w457, y=w458) -> (x != y?=w453:bool)
                n224 = Or(x=w453, y=w454) -> (x .or. y?=w452:bool)
              }
              n225 = Path To String(path=w437) -> (string=w443:string[])
              n226 = Bundle By Name(cluster=T16 {"XYZ Positions"=[], "File Paths"=[]} ("Marked Positions"), "XYZ Positions"=w434, "File Paths"=w443) -> (w442:T16)
              n227 = Flatten To JSON(anything=w442) -> (JSON string=w441:string, 11:w439:errorcluster)  [unwired: 2 in]
              n228 = Write to Text File(file (use dialog)=w433, text=w441, error in=w439) -> (refnum out=w440:refnum<file>, error out=w438:errorcluster)  [unwired: 1 in, 1 out]
              n229 = Close File(refnum=w440, error in=w438) -> ()  [unwired: 2 out]
            }
            frame "Clear All" {
              n230 = Flatten To JSON(anything=T16 {"XYZ Positions"=[], "File Paths"=[]} ("Marked Positions")) -> (JSON string=w465:string, 11:w463:errorcluster)  [unwired: 2 in]
              n231 = Write to Text File(file (use dialog)=w460, text=w465, error in=w463) -> (refnum out=w464:refnum<file>, error out=w462:errorcluster)  [unwired: 1 in, 1 out]
              n232 = Close File(refnum=w464, error in=w462) -> ()  [unwired: 2 out]
              n233 = Initialize Array(path "", 0 ("dimension size")) -> (w468:path[])
            }
            frame "Quit" {
              n234 = case shown="No Error" w474 {
                tunnel: w476 -> [w480 _]
                tunnel: w475 -> [w479 _]
                frame No Error {
                  n235 = Release Notifier(notifier=w480) -> ()  [unwired: 2 in, 3 out]
                  n236 = Release Notifier(notifier=w479) -> ()  [unwired: 2 in, 3 out]
                }
                frame Error {
                }
              }
              n237 = Release Notifier(notifier=w473) -> ()  [unwired: 2 in, 3 out]
            }
          }
        }
      }
      n238 = local write "Quit"(w99) -> ()
    }
    frame Error {
      w584 = "\r"
      n239 = Release Notifier(notifier=w586, error in (no error)=w585) -> (error out=w582:errorcluster)  [unwired: 1 in, 2 out]
      n240 = Unbundle By Name(w582) -> ("source"=w581:string)
      n241 = Concatenate Strings("Image Multiple Areas had a startup error.", w584, w584, w581) -> (w580:string)
      n242 = One Button Dialog(message=w580) -> ()  [unwired: 1 in, 1 out]
    }
  }
  n243 = control-ref of="This VI"() -> (w21:refnum<vi>)
  n244 = property class="VI"(reference=w21) -> (reference out=w30:refnum<vi>, "Panel"=w22:refnum<vi>)  [unwired: 1 in, 1 out]
  n245 = property class="Pnl"(reference=w22) -> ("Decos[]"=w20:refnum<vi>[], "Panes[]"=w26:refnum<vi>[])  [unwired: 1 in, 2 out]
  n246 = Array Size(array=w20) -> (size(s)=w18:i32)
  n247 = Decrement(x=w18) -> (x-1=w19:i32)
  n248 = Index Array(array=w26, index=0) -> (element=w25:refnum<vi>)
  n249 = Index Array(array=w20, index=w19) -> (element=w28:refnum<vi>)
  n250 = property class="VI"(reference=w30) -> (reference out=w32:refnum<vi>, "Front Panel.PanelBounds"=w33:T20)  [unwired: 1 in, 1 out]
  n251 = property class="Decor"(reference=w28) -> ("Bounds"=w31:T21)  [unwired: 1 in, 2 out]
  n252 = property class="Pane"(reference=w25, "Origin"=T6 {"Horizontal"=0, "Vertical"=0}, "HorizScrollbarVisibility"=w29, "VertScrollbarVisibility"=w29) -> ()  [unwired: 1 in, 2 out]
  n253 = Unbundle By Name(w31) -> ("Width"=w36:u32, "Height"=w39:u32)
  n254 = control-ref of="Quit"() -> (w23:refnum<vi>)
  n255 = To Word Integer(number=w36) -> (16bit integer=w38:i16)
  n256 = To Word Integer(number=w39) -> ()  [unwired: 1 out]
  n257 = property class="Bool (strict)"(reference=w23) -> ("Height"=w41:u32, "Top"=w42:i32)  [unwired: 1 in, 2 out]
  n258 = Unbundle By Name(w33) -> ("Left"=w35:i16, "Top"=w46:i16)
  n259 = To Word Integer(number=w41) -> (16bit integer=w44:i16)
  n260 = To Word Integer(number=w42) -> (16bit integer=w45:i16)
  n261 = Add(x=w35, y=w38) -> (x+y=w37:i16)
  n262 = Compound Arithmetic op=ADD(w46, w44, w45, i16 12 ("y")) -> (w40:i16)
  n263 = Bundle By Name(cluster=w33, "Right"=w37, "Bottom"=w40) -> (w34:T20)
  n264 = property class="VI"(reference=w32, "Front Panel.PanelBounds"=w34) -> ()  [unwired: 1 in, 2 out]
